vi "Parameter XML Write (AIM-1533).vi"(6 "hw configuration":T1, 8 "error in":errorcluster caption="error out", 9 "hardwareChannel":i32, 10 "aim1553_cluster":T2, 11 "parameter file in":refnum<k24>) -> (0 "error out":errorcluster, 3 "parameter file out":refnum<k24>)   [LabVIEW 2020]
uses:
  _controls/aim1553_cluster.ctl
  _controls/aim1553_messages.ctl
  _controls/1553_Parameters_key.ctl
  _controls/1553_Parameters.ctl
  _controls/1553_minorFrames.ctl
  C:/Users/Administrator/Desktop/GIT/Ballard-Arinc-429-XML-Generator/Source/Assemblies/Aim_1553_Parameter_ni/bin/Debug/AIM_1553_Parameter_ni.dll
  Assemblies/Aim_1553_Parameter_ni/bin/Debug/AIM_1553_Parameter_ni.dll
  _controls/aim1553_RT_list.ctl
  Libraries/Aim_1553_Parameter_ni/_tyedefs/message_type.ctl
  Libraries/Aim_1553_Parameter_ni/_tyedefs/messageAddress_type.ctl
  Libraries/Aim_1553_Parameter_ni/_tyedefs/parameter_type.ctl
  Libraries/Aim_1553_Parameter_ni/AIM_1553_Parameter_ni.lvlib
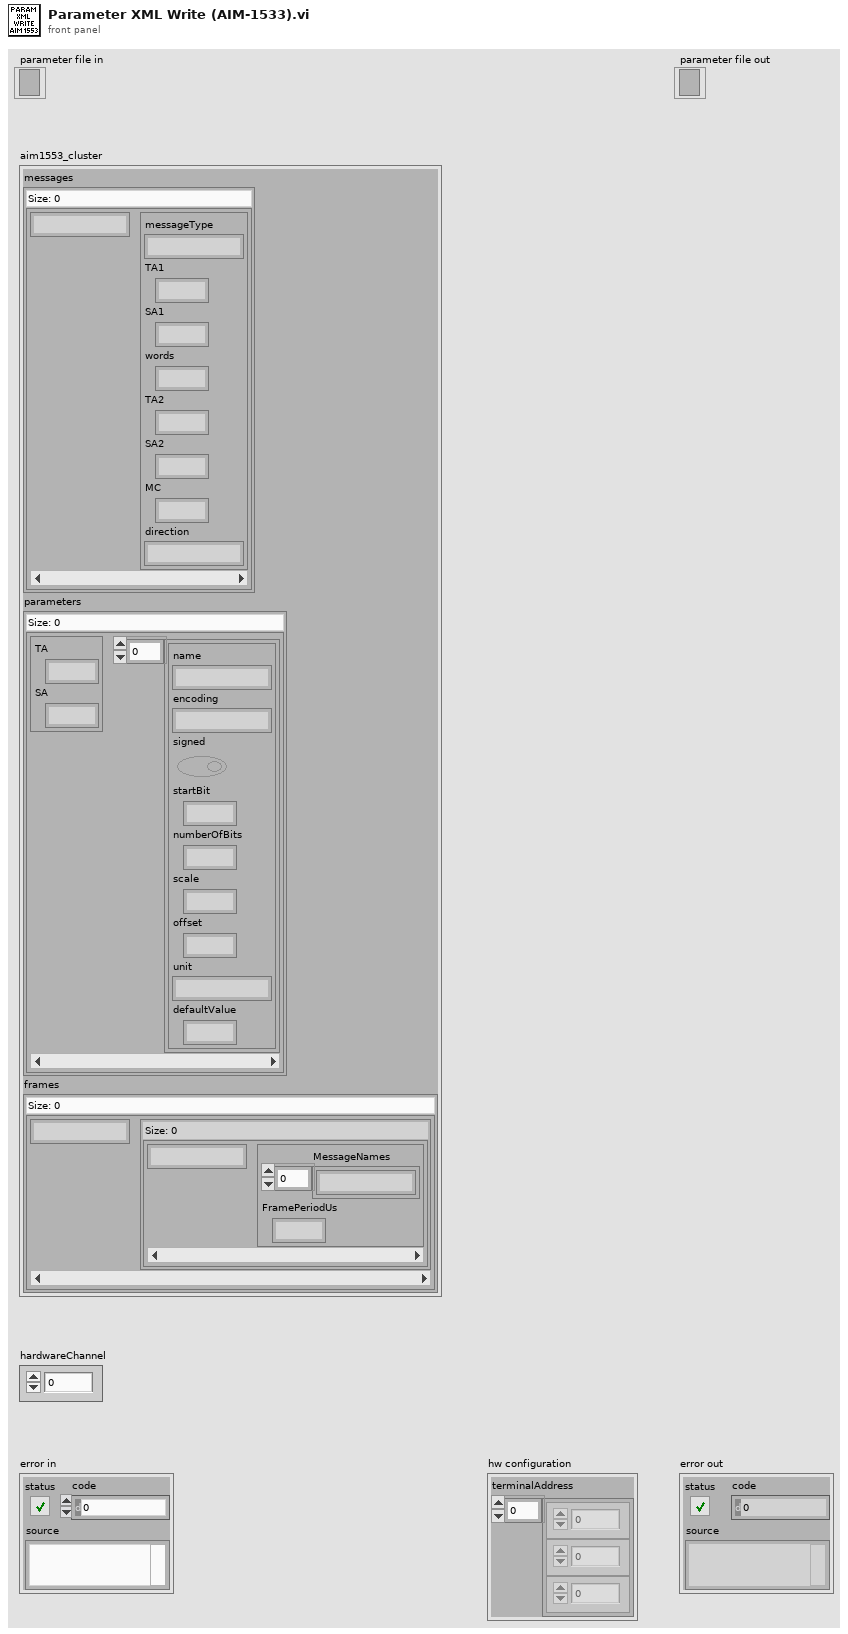
[diagram p1: front panel]
types:
  T1 = typedef "aim1553_RT_list.ctl" = cluster{"terminalAddress":i32[]}
  T2 = typedef "aim1553_cluster.ctl" = cluster{"messages":map{string, T3}, "parameters":map{T4, T5[]}, "frames":map{string, map{string, T6}}}
  T3 = typedef "aim1553_messages.ctl" = cluster{"messageType":string, "TA1":i32, "SA1":i32, "words":i32, "TA2":i32, "SA2":i32, "MC":i32, "direction":string}
  T4 = typedef "1553_Parameters_key.ctl" = cluster{"TA":i32, "SA":i32}
  T5 = typedef "1553_Parameters.ctl" = cluster{"name":string, "encoding":string, "signed":bool, "startBit":i32, "numberOfBits":i32, "scale":dbl, "offset":dbl, "unit":string, "defaultValue":dbl}
  T6 = typedef "1553_minorFrames.ctl" = cluster{"MessageNames":string[], "FramePeriodUs":i32}
  T7 = typedef "AIM_1553_Parameter_ni.lvlib/message_type.ctl" = cluster{"name":string, "numberOfWords":i32, "modeCode":i32, "messageType":i32, "createTimestampChannel":bool, "modeCodeSpecified":bool}
  T8 = typedef "AIM_1553_Parameter_ni.lvlib/parameter_type.ctl" = cluster{"defaultValue":dbl, "encoding":i32, "name":string, "numberOfBits":i32, "offset":dbl, "scale":dbl, "signed":bool, "startBit":i32, "unit":string}
  T9 = typedef "AIM_1553_Parameter_ni.lvlib/messageAddress_type.ctl" = cluster{"direction":i32, "subAddress":i32, "terminalAddress":i32}
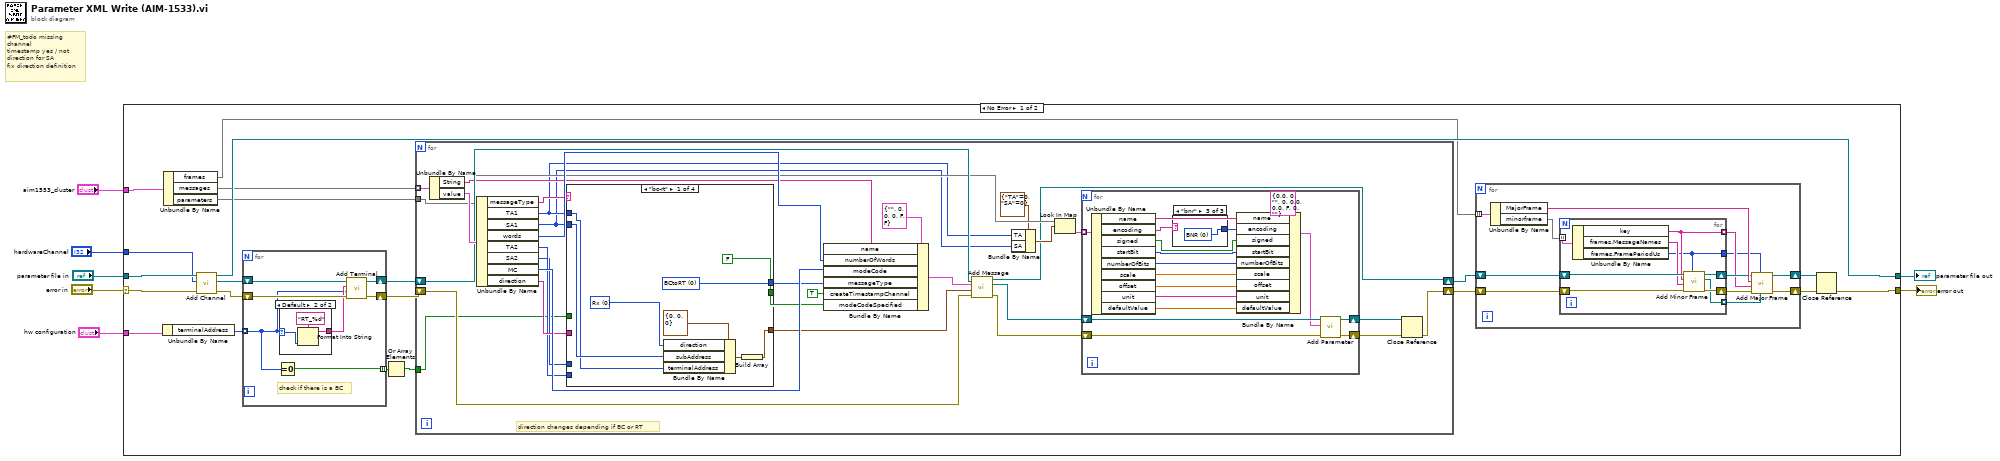
[diagram p0: block diagram]
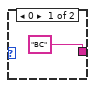
[diagram p2: hidden frame]
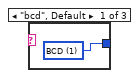
[diagram p3: hidden frame]
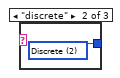
[diagram p4: hidden frame]
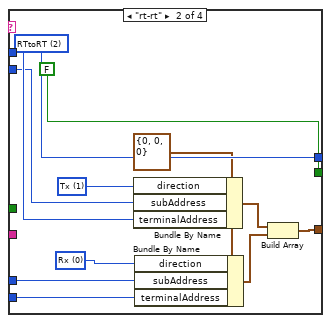
[diagram p5: hidden frame]
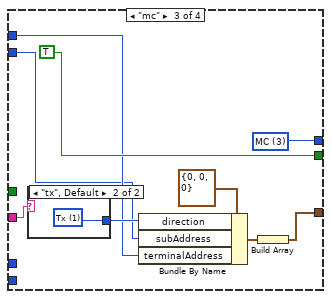
[diagram p6: hidden frame]
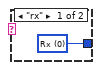
[diagram p7: hidden frame]
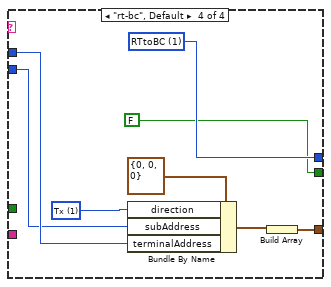
[diagram p8: hidden frame]
diagram:
  # "#FM_todo missing \nchannel\ntimestamp yes / not\ndirection for SA\nfix direction definition"
  n1 = case shown="No Error" "error in" {
    selector: "error in" -> [w27 w151]
    tunnel: "aim1553_cluster" -> [w26 _]
    tunnel: "parameter file in" -> [w28 w150]
    tunnel: [w24 w151] -> w4
    tunnel: [w25 w150] -> w3
    tunnel: "hw configuration" -> [w23 _]
    tunnel: "hardwareChannel" -> [w22 _]
    frame No Error {
      n2 = Unbundle By Name(w23) -> ("terminalAddress"=w10:i32[])
      n3 = Unbundle By Name(w26) -> ("frames"=w11:map{string, map{string, T6}}, "messages"=w21:map{string, T3}, "parameters"=w20:map{T4, T5[]})
      n4 = call "Add Channel.vi"("error in"=w27, "hardwareChannel"=w22, "parameter file in"=w28) -> ("error out"=w19:errorcluster, "new channel"=w18:refnum<k24>, "parameter file out"=w25:refnum<k24>)  [unwired: 6 in]
      n5 = for {
        shift-right: [w33] -> w17
        shift-left: w19 -> [w35]
        shift-right: [w32] -> w16
        shift-left: w18 -> [w34]
        tunnel: w10 -> [w30] mode=indexing
        tunnel: [w29] -> w9 mode=indexing
        # "check if there is a BC"
        n6 = Equal To 0?(x=w30) -> (x = 0?=w29:bool)
        n7 = case shown="Default" w30 {
          selector: w30 -> [_ w38]
          tunnel: ["BC" ("BC") w39] -> w31
          frame 0 {
          }
          frame Default {
            n8 = Format Into String(format string="RT_%d", w38) -> (resulting string=w39:string)  [unwired: 2 in, 1 out]
          }
        }
        n9 = call "Add Terminal.vi"("error in"=w35, "terminalAddress"=w30, "name"=w31, "channel in"=w34) -> ("error out"=w33:errorcluster, "channel out"=w32:refnum<k24>)  [unwired: 5 in, 1 out]
      }
      n10 = Or Array Elements(Boolean array=w9) -> (logical OR=w8:bool)
      n11 = for {
        tunnel: w21 -> [w90] mode=indexing
        tunnel: w20 -> [w70]
        shift-right: [w62] -> w15
        shift-left: w16 -> [w87]
        shift-right: [w63] -> w14
        shift-left: w17 -> [w77]
        tunnel: w8 -> [w61]
        # "direction changes depending if BC or RT"
        n12 = Unbundle By Name(w90) -> ("String"=w69:string, "value"=w89:T3)
        n13 = Unbundle By Name(w89) -> ("messageType"=w84:string, "TA1"=w66:i32, "SA1"=w65:i32, "words"=w85:i32, "TA2"=w72:i32, "SA2"=w71:i32, "MC"=w83:i32, "direction"=w79:string)
        n14 = case shown="\"bc-rt\"" w84 {
          tunnel: [w118 w130 w139 w149] -> w81
          tunnel: [FALSE FALSE TRUE FALSE] -> w80
          tunnel: w79 -> [_ _ w135 _]
          tunnel: w66 -> [w114 w122 w133 w145]
          tunnel: w65 -> [w115 w121 w132 w144]
          tunnel: [w112 w124 w131 w142] -> w78
          tunnel: w72 -> [_ w120 _ _]
          tunnel: w71 -> [_ w119 _ _]
          tunnel: w61 -> [_ _ _ _]
          frame "bc-rt" {
            w111 = 0 items=["Rx", "Tx"] ("direction")
            w118 = 0 items=["BCtoRT", "RTtoBC", "RTtoRT", "MC"] ("messageType")
            n15 = Bundle By Name(cluster=T9 {"direction"=0, "subAddress"=0, "terminalAddress"=0} ("messageAddress"), "direction"=w111, "subAddress"=w115, "terminalAddress"=w114) -> (w113:T9)
            n16 = Build Array(w113) -> (w112:T9[])
          }
          frame "rt-rt" {
            w123 = 0 items=["Rx", "Tx"] ("direction")
            w128 = 1 items=["Rx", "Tx"] ("direction")
            w125 = T9 {"direction"=0, "subAddress"=0, "terminalAddress"=0} ("messageAddress")
            w130 = 2 items=["BCtoRT", "RTtoBC", "RTtoRT", "MC"] ("messageType")
            n17 = Bundle By Name(cluster=w125, "direction"=w128, "subAddress"=w121, "terminalAddress"=w122) -> (w127:T9)
            n18 = Bundle By Name(cluster=w125, "direction"=w123, "subAddress"=w119, "terminalAddress"=w120) -> (w126:T9)
            n19 = Build Array(w127, w126) -> (w124:T9[])
          }
          frame "mc" {
            w139 = 3 items=["BCtoRT", "RTtoBC", "RTtoRT", "MC"] ("messageType")
            n20 = case shown="\"tx\", Default" w135 {
              tunnel: [w140 w141] -> w134
              frame "rx" {
                w140 = 0 items=["Rx", "Tx"] ("direction")
              }
              frame "tx", Default {
                w141 = 1 items=["Rx", "Tx"] ("direction")
              }
            }
            n21 = Bundle By Name(cluster=T9 {"direction"=0, "subAddress"=0, "terminalAddress"=0} ("messageAddress"), "direction"=w134, "subAddress"=w132, "terminalAddress"=w133) -> (w136:T9)
            n22 = Build Array(w136) -> (w131:T9[])
          }
          frame "rt-bc", Default {
            w146 = 1 items=["Rx", "Tx"] ("direction")
            w149 = 1 items=["BCtoRT", "RTtoBC", "RTtoRT", "MC"] ("messageType")
            n23 = Bundle By Name(cluster=T9 {"direction"=0, "subAddress"=0, "terminalAddress"=0} ("messageAddress"), "direction"=w146, "subAddress"=w144, "terminalAddress"=w145) -> (w143:T9)
            n24 = Build Array(w143) -> (w142:T9[])
          }
        }
        n25 = Bundle By Name(cluster=T7 {"name"="", "numberOfWords"=0, "modeCode"=0, "messageType"=0, "createTimestampChannel"=FALSE, "modeCodeSpecified"=FALSE} ("message configuration"), "name"=w69, "numberOfWords"=w85, "modeCode"=w83, "messageType"=w81, "createTimestampChannel"=TRUE, "modeCodeSpecified"=w80) -> (w86:T7)
        n26 = call "Add Message.vi"("error in"=w77, "messageAddresses"=w78, "message configuration"=w86, "channel in"=w87) -> ("error out"=w76:errorcluster, "new message"=w75:refnum<k24>, "channel out"=w62:refnum<k24>)  [unwired: 5 in]
        n27 = Bundle By Name(cluster=T4 {"TA"=0, "SA"=0} ("key"), "TA"=w66, "SA"=w65) -> (w67:T4)
        n28 = Look In Map(map=w70, key=w67) -> (value=w64:T5[])  [unwired: 1 in, 1 out]
        n29 = for {
          shift-right: [w104] -> w73
          shift-left: w76 -> [w107]
          shift-right: [w105] -> w74
          shift-left: w75 -> [w106]
          tunnel: w64 -> [w102] mode=indexing
          n30 = Unbundle By Name(w102) -> ("name"=w100:string, "encoding"=w99:string, "signed"=w97:bool, "startBit"=w96:i32, "numberOfBits"=w95:i32, "scale"=w94:dbl, "offset"=w93:dbl, "unit"=w92:string, "defaultValue"=w91:dbl)
          n31 = case shown="\"bnr\"" w99 {
            tunnel: [w108 w109 w110] -> w98
            frame "bcd", Default {
              w108 = 1 items=["BNR", "BCD", "Discrete"] ("encoding")
            }
            frame "discrete" {
              w109 = 2 items=["BNR", "BCD", "Discrete"] ("encoding")
            }
            frame "bnr" {
              w110 = 0 items=["BNR", "BCD", "Discrete"] ("encoding")
            }
          }
          n32 = Bundle By Name(cluster=T8 {"defaultValue"=0.0, "encoding"=0, "name"="", "numberOfBits"=0, "offset"=0.0, "scale"=0.0, "signed"=FALSE, "startBit"=0, "unit"=""} ("parameter configuration"), "name"=w100, "encoding"=w98, "signed"=w97, "startBit"=w96, "numberOfBits"=w95, "scale"=w94, "offset"=w93, "unit"=w92, "defaultValue"=w91) -> (w101:T8)
          n33 = call "Add Parameter.vi"("error in"=w107, "parameter configuration"=w101, "message in"=w106) -> ("error out"=w104:errorcluster, "message out"=w105:refnum<k24>)  [unwired: 6 in, 1 out]
        }
        n34 = Close Reference(reference=w74, error in (no error)=w73) -> (error out=w63:errorcluster)
      }
      n35 = for {
        shift-right: [w51] -> w13
        shift-left: w15 -> [w47]
        shift-right: [w50] -> w12
        shift-left: w14 -> [w45]
        tunnel: w11 -> [w49] mode=indexing
        n36 = Unbundle By Name(w49) -> ("MajorFrame"=w48:string, "minorframe"=w43:map{string, T6})
        n37 = for {
          shift-right: [w59] -> w46
          shift-left: w47 -> [w57]
          shift-right: [w58] -> w44
          shift-left: w45 -> [w56]
          tunnel: w43 -> [w60] mode=indexing
          tunnel: [w54] -> w42 mode=indexing
          tunnel: [w53] -> w41
          tunnel: [w52] -> w40 mode=indexing
          n38 = Unbundle By Name(w60) -> ("key"=w54:string, "frames.MessageNames"=w55:string[], "frames.FramePeriodUs"=w53:i32)
          n39 = call "Add Minor Frame.vi"("minorFramePeriod"=w53, "error in"=w56, "messageRefs"=w55, "name"=w54, "channel in"=w57) -> ("error out"=w58:errorcluster, "new minor frame"=w52:refnum<k24>, "channel out"=w59:refnum<k24>)  [unwired: 4 in]
        }
        n40 = call "Add Major Frame.vi"("minorFrameRefs"=w40, "minorFramePeriod"=w41, "error in"=w44, "minorFrameNames"=w42, "name"=w48, "channel in"=w46) -> ("error out"=w50:errorcluster, "channel out"=w51:refnum<k24>)  [unwired: 3 in, 1 out]
      }
      n41 = Close Reference(reference=w13, error in (no error)=w12) -> (error out=w24:errorcluster)
    }
    frame Error {
    }
  }
  "error out" <- w4
  "parameter file out" <- w3
